vi "Arreglo_case.vi"() -> ()   [LabVIEW 2026]
panel:
  in  "ORIGINAL":dbl[][](array[numeric])
  in  "Tab Control":enum32{"FILA", "COLUMNA", "CELDA"}(tab)
  in  "FILA":i16
  out "FILA MODIFICADA":dbl[][](array[numeric])
  in  "NUEVA FILA":dbl[](array[numeric])
  in  "COLUMNA":i16
  in  "NUEVA COLUMNA":dbl[](array[numeric])
  out "COLUMNA MODIFICADA":dbl[][](array[numeric])
  in  "FILA":i16
  in  "COLUMNA":i16
  in  "NUEVA CELDA":dbl
  out "CELDA MODIFICADA":dbl[][](array[numeric])
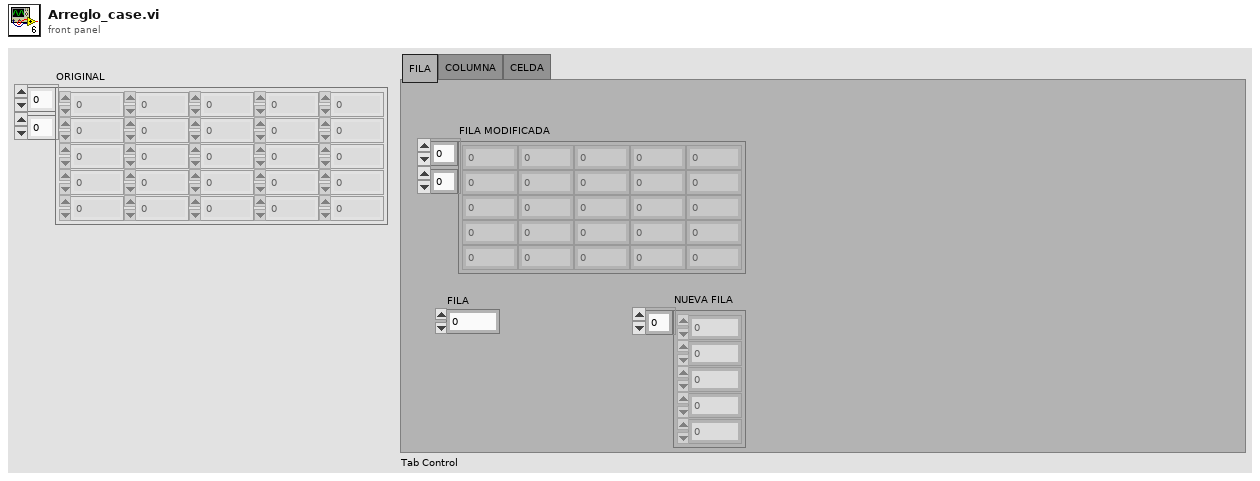
[diagram p1: front panel]
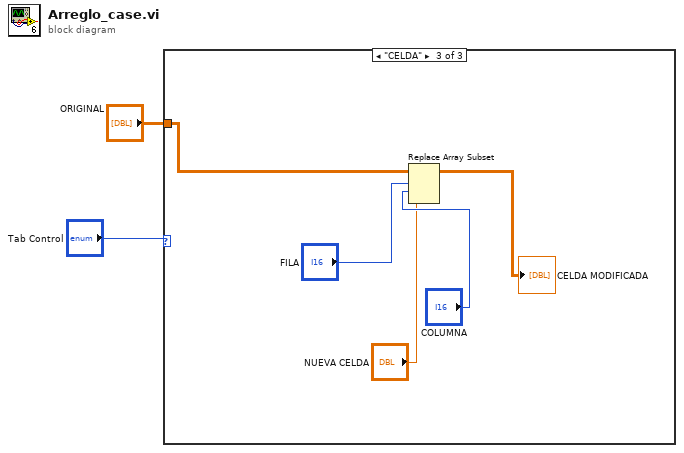
[diagram p0: block diagram]
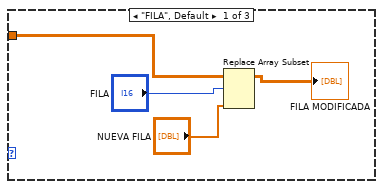
[diagram p2: hidden frame]
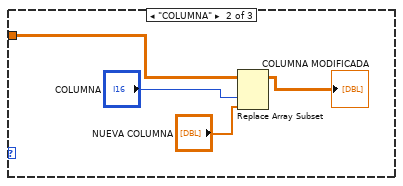
[diagram p3: hidden frame]
diagram:
  n1 = case shown="\"CELDA\"" "Tab Control" {
    tunnel: "ORIGINAL" -> [w3 w9 w15]
    frame "FILA", Default {
      n2 = Replace Array Subset(array=w3, new element="NUEVA FILA", index (row)="FILA") -> (→"FILA MODIFICADA":dbl[][])  [unwired: 1 in]
    }
    frame "COLUMNA" {
      n3 = Replace Array Subset(array=w9, new element="NUEVA COLUMNA", index (col)="COLUMNA") -> (→"COLUMNA MODIFICADA":dbl[][])  [unwired: 1 in]
    }
    frame "CELDA" {
      n4 = Replace Array Subset(array=w15, new element="NUEVA CELDA", index (row)="FILA", index (col)="COLUMNA") -> (→"CELDA MODIFICADA":dbl[][])
    }
  }
